vi "Move.vi"(8 "error in":errorcluster, 9 "Target":path, 10 "Source":path, 11 "IFile Manager in":refnum<class "Mock IFile Manager.lvclass">) -> (0 "error out":errorcluster, 3 "IFile Manager out":refnum<class "Mock IFile Manager.lvclass">)   [LabVIEW 2026, in "Mock IFile Manager.lvclass"]
doc: "Move (aka rename) source to target."
uses:
  Mock IFile Manager.lvclass
  C:/Program Files/National Instruments/LabVIEW 2026/vi.lib/Astemes/LMock/Mock.lvclass
  Mock IFile Manager.lvclass/Mock IFile Manager.ctl
  <vilib>/Astemes/LMock/Mock.lvclass
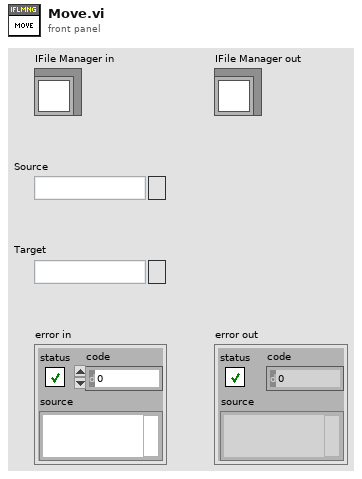
[diagram p1: front panel]
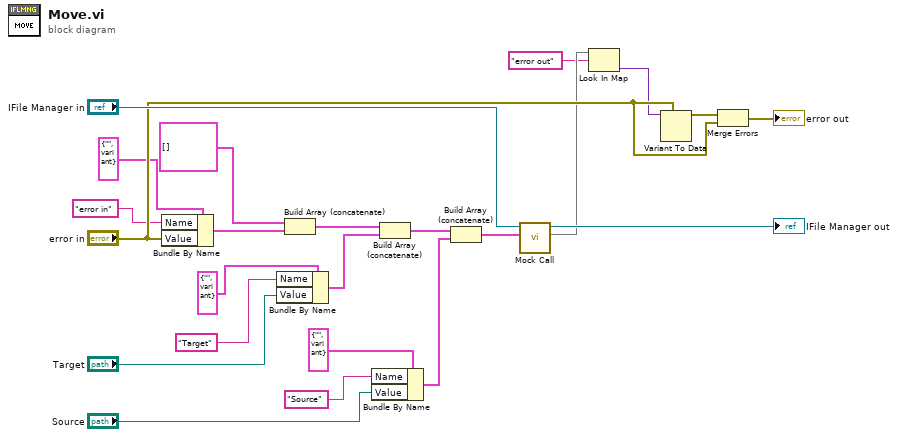
[diagram p0: block diagram]
diagram:
  n1 = Bundle By Name(cluster=cluster{"Name":string, "Value":variant} {"Name"="", "Value"=variant} ("element"), "Name"="error in", "Value"="error in") -> (w5:cluster{"Name":string, "Value":variant})
  n2 = Bundle By Name(cluster=cluster{"Name":string, "Value":variant} {"Name"="", "Value"=variant} ("element"), "Name"="Target", "Value"="Target") -> (w3:cluster{"Name":string, "Value":variant})
  n3 = Build Array (concatenate)(cluster{"Name":string, "Value":variant}[] [] ("Control Values"), w5) -> (w14:cluster{"Name":string, "Value":variant}[])
  n4 = Bundle By Name(cluster=cluster{"Name":string, "Value":variant} {"Name"="", "Value"=variant} ("element"), "Name"="Source", "Value"="Source") -> (w1:cluster{"Name":string, "Value":variant})
  n5 = Build Array (concatenate)(w14, w3) -> (w17:cluster{"Name":string, "Value":variant}[])
  n6 = Build Array (concatenate)(w17, w1) -> (w20:cluster{"Name":string, "Value":variant}[])
  n7 = call <vilib>:"Mock Call.vi"("Control Values"=w20, "Mock In"="IFile Manager in") -> ("Return Values"=w12:map{string, variant}, "Mock Out"=→"IFile Manager out":refnum<class "Mock IFile Manager.lvclass">)  [unwired: 8 in]
  n8 = Look In Map(map=w12, key="error out") -> (value=w10:variant)  [unwired: 1 in, 1 out]
  n9 = Variant To Data(type="error in", Variant=w10) -> (data=w9:errorcluster)  [unwired: 1 in, 1 out]
  n10 = Merge Errors(w9, "error in") -> (→"error out":errorcluster)
